vi "MoveNode.vi"(8 "error in":errorcluster, 9 "index":i32, 10 "new parent":T1, 11 "node":T1) -> (0 "error out":errorcluster)   [LabVIEW 2014, in "NISE_CEF_TreeControl.lvlib"]
doc: "Moves a node to a new parretn updating the reference in the 3 nodes (child, old parent and new parent)."
uses:
  NISE_CEF_TreeControl.lvlib
  Node/NodeRef.ctl
  Node/NISE_CEF_Node.lvclass
  Node/NISE_CEF_Node.lvclass/NISE_CEF_Node.ctl
  Node/ReadParent.vi
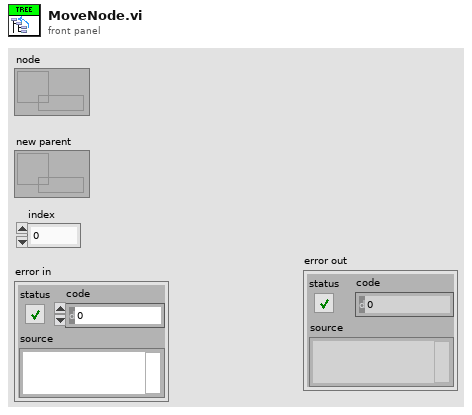
[diagram p1: front panel]
types:
  T1 = typedef "NISE_CEF_Node.lvclass/NodeRef.ctl" = refnum<data-value>
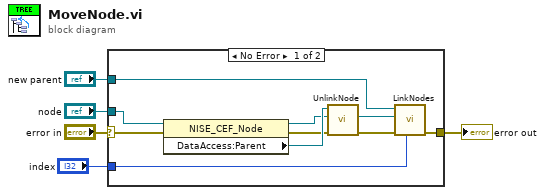
[diagram p0: block diagram]
diagram:
  n1 = case shown="No Error" "error in" {
    selector: "error in" -> [w7 w16]
    tunnel: [w9 w16] -> w4
    tunnel: "node" -> [w14 _]
    tunnel: "new parent" -> [w10 _]
    tunnel: "index" -> [w6 _]
    frame No Error {
      n2 = property class="NISE_CEF_Node"(reference=w14, error in=w7) -> (reference out=w11:T1, error out=w8:errorcluster, "DataAccess:Parent"=w15:T1)
      n3 = call "UnlinkNode.vi"("error in"=w8, "child in"=w11, "parent in"=w15) -> ("error out"=w13:errorcluster, "child out"=w12:T1)  [unwired: 6 in, 1 out]
      n4 = call "LinkNodes.vi"("index"=w6, "error in"=w13, "child in"=w12, "parent in"=w10) -> ("error out"=w9:errorcluster)  [unwired: 5 in, 2 out]
    }
    frame Error {
    }
  }
  "error out" <- w4
